vi "InstrumentStudio Screenshot Capture.vi"(8 "error in":errorcluster, 10 "Base File Name (*.bmp)":string="InstrStudio_Screenshot.bmp", 11 "Output Folder to Save Screenshot":path=path "C:/Temp") -> (0 "error out":errorcluster, 3 "Save Image Successful?":bool)   [LabVIEW 2025, in "Screenshot Utility.lvlib"]
doc: "This VI captures a screenshot of the InstrumentStudio window using Windows GDI APIs (works even if hidden).\n\nFor saving the screenshot of InstrumentStudio:\n • Provide a valid output folder and base file name.\n • Ensure InstrumentStudio is running with required SFPs loaded (window must exist).\n • Automatically appends a timestamp to the file name before saving.\n • Works only on Windows; capture fails if the window is not found or title is incorrect."
uses:
  Screenshot Utility.lvlib
  User32.dll
  GDI32.DLL
panel:
  # "This VI captures a screenshot of the InstrumentStudio window using Windows GDI APIs (works even if hidden).\n\nFor saving the screenshot of InstrumentStudio:\n • Provide a valid output folder and base file name.\n • Ensure InstrumentStudio is running with required SFPs loaded (window must exist).\n • Automatically appends a timestamp to the file name before saving.\n • Works only on Windows; capture fails if the window is not found or title is incorrect."
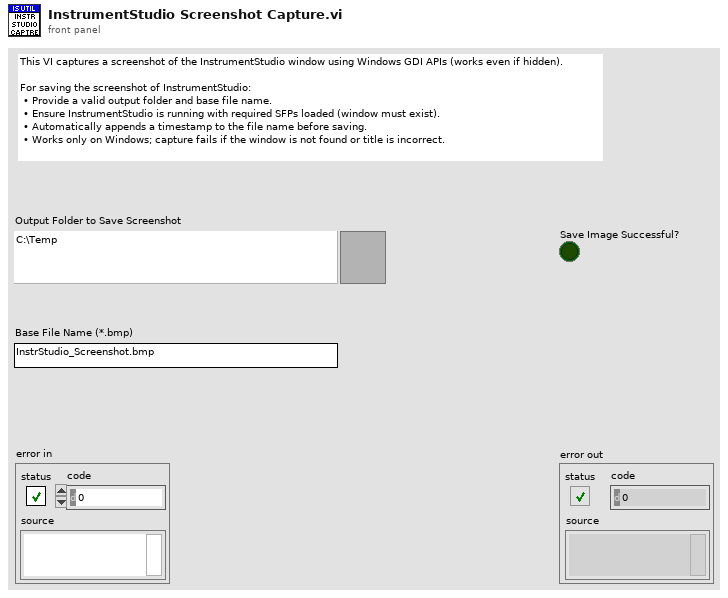
[diagram p1: front panel]
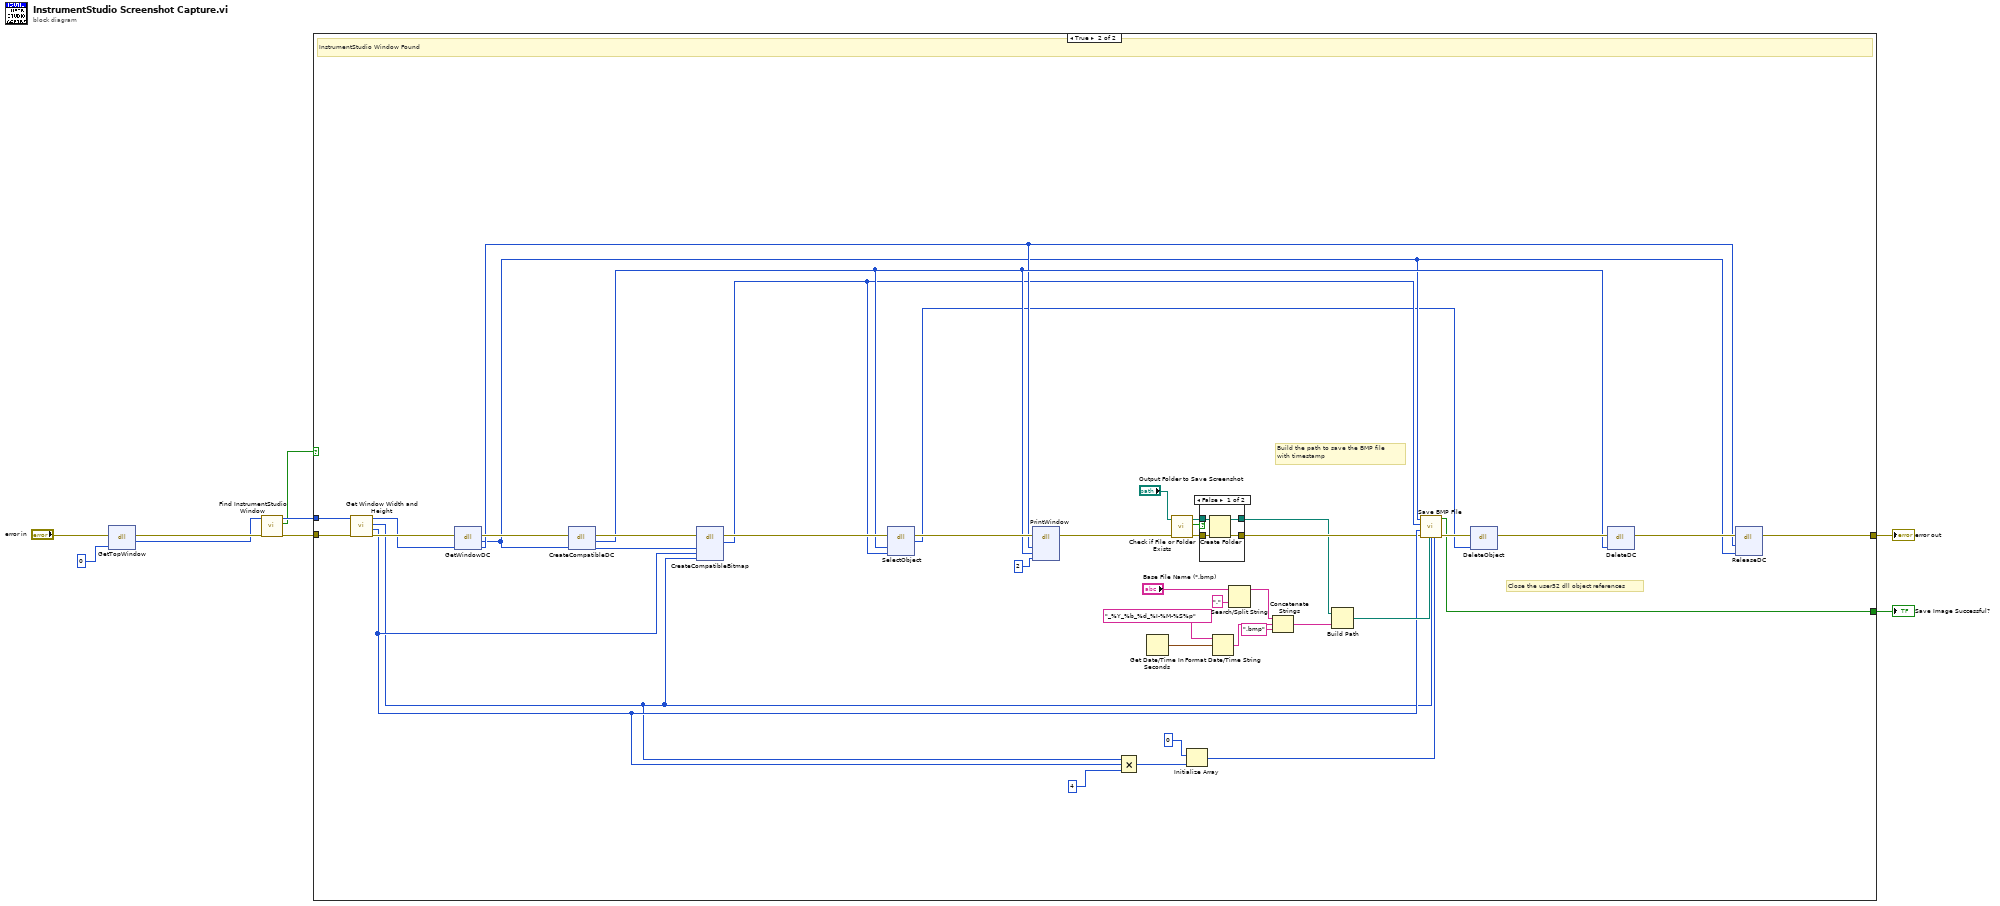
[diagram p0: block diagram]
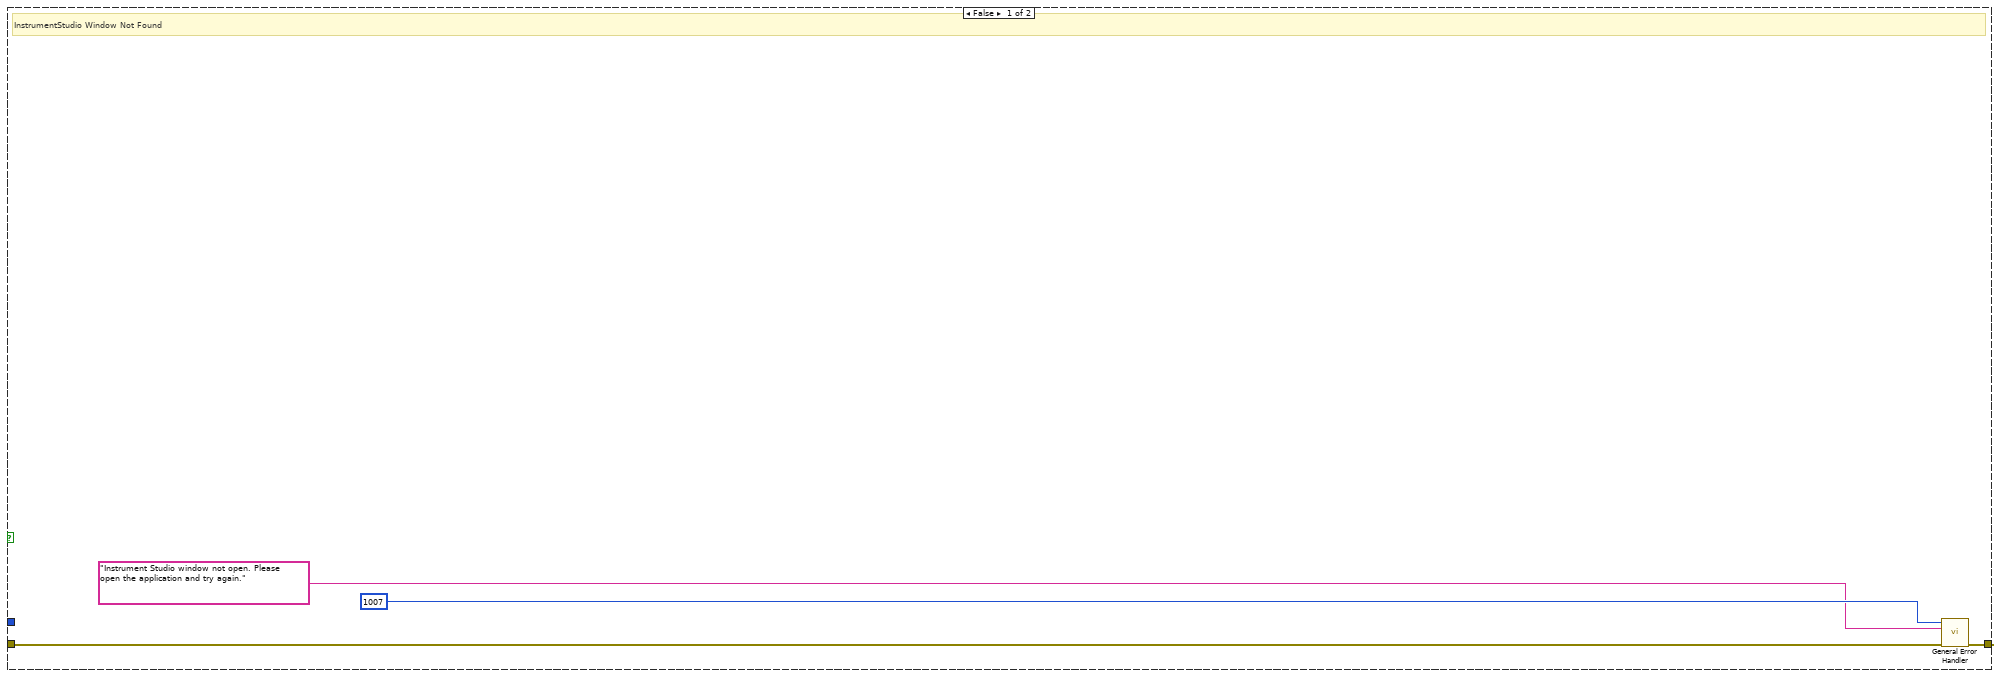
[diagram p2: hidden frame]
diagram:
  n1 = dll-call lib="USER32.DLL" fn="GetTopWindow"(error in="error in", "hWnd"=u32 0) -> (error out=w8:errorcluster, "return"=w6:u32)  [unwired: 2 in, 2 out]
  n2 = call "Find InstrumentStudio Window.vi"("error in"=w8, "Top Window"=w6) -> ("error out"=w3:errorcluster, "IS Window Found?"=w2:bool, "hWnd"=w4:u32)  [unwired: 7 in]
  n3 = case shown="True" w2 {
    tunnel: [w12 w45] -> w5
    tunnel: w4 -> [_ w21]
    tunnel: w3 -> [w13 w22]
    tunnel: [_ w23] -> w1
    frame False {
      # "InstrumentStudio Window Not Found"
      n4 = call <vilib>:"General Error Handler.vi"("[error code] (0)"=1007, "[error source] (\" \")"="Instrument Studio window not open. Please open the application and try again." ("[error source] (\" \")"), "error in (no error)"=w13) -> ("error out"=w12:errorcluster)  [unwired: 8 in, 4 out]
    }
    frame True {
      # "Close the user32 dll object references"
      # "Build the path to save the BMP file \nwith timestamp"
      # "InstrumentStudio Window Found"
      n5 = call "Get Window Width and Height.vi"("error in"=w22, "hWnd in"=w21) -> ("error out"=w41:errorcluster, "Width"=w25:i32, "Height"=w24:i32, "hWnd out"=w39:u32)  [unwired: 6 in]
      n6 = dll-call lib="USER32.DLL" fn="GetWindowDC"(error in=w41, "hWnd"=w39) -> (error out=w55:errorcluster, "return"=w43:u32, "hWnd"=w44:u32)  [unwired: 2 in, 1 out]
      n7 = dll-call lib="GDI32.DLL" fn="CreateCompatibleDC"(error in=w55, "hdc"=w43) -> (error out=w47:errorcluster, "return"=w46:u32, "hdc"=w54:u32)  [unwired: 2 in, 1 out]
      n8 = dll-call lib="GDI32.DLL" fn="CreateCompatibleBitmap"(error in=w47, "hdc"=w54, "cx"=w25, "cy"=w24) -> (error out=w53:errorcluster, "return"=w37:u32)  [unwired: 2 in, 4 out]
      n9 = dll-call lib="GDI32.DLL" fn="SelectObject"(error in=w53, "hdc"=w46, "h"=w37) -> (error out=w52:errorcluster, "return"=w35:u32)  [unwired: 2 in, 3 out]
      n10 = dll-call lib="USER32.DLL" fn="PrintWindow"(error in=w52, "hWnd"=w44, "hdcBlt"=w46, "nFlags"=u32 2) -> (error out=w17:errorcluster)  [unwired: 2 in, 5 out]
      n11 = Compound Arithmetic op=MULTIPLY(w24, w25, 4 ("value")) -> (w42:i32)
      n12 = Get Date/Time In Seconds() -> (seconds since 1Jan1904=w34:timestamp)
      n13 = call <vilib>:"Check if File or Folder Exists.vi"("error in (no error)"=w17, "path"="Output Folder to Save Screenshot") -> ("error out"=w20:errorcluster, "file or folder exists?"=w18:bool, "dup path"=w19:path)  [unwired: 7 in]
      n14 = Initialize Array(u8 0 ("element"), w42) -> (w38:u8[])
      n15 = case shown="False" w18 {
        tunnel: [w59 w60] -> w16
        tunnel: [w58 w61] -> w14
        tunnel: w20 -> [w57 w60]
        tunnel: w19 -> [w56 w61]
        frame False {
          n16 = Create Folder(path (use dialog)=w56, error in=w57) -> (created path=w58:path, error out=w59:errorcluster)  [unwired: 1 in, 1 out]
        }
        frame True {
        }
      }
      n17 = Format Date/Time String(time format string (%c)="_%Y_%b_%d_%I-%M-%S%p", seconds (now)=w34) -> (date/time string=w29:string)  [unwired: 1 in]
      n18 = Search/Split String(string="Base File Name (*.bmp)", search string/char (-)=".") -> (substring before match=w30:string)  [unwired: 1 in, 2 out]
      n19 = Concatenate Strings(w30, w29, ".bmp" ("string")) -> (w27:string)
      n20 = Build Path(base path=w14, name or relative path=w27) -> (appended path=w26:path)
      n21 = call "Save BMP File.vi"("lpvBits Array"=w38, "Height"=w24, "Path to BMP file"=w26, "error in"=w16, "Width"=w25, "hbm"=w37, "hdc"=w43) -> ("error out"=w36:errorcluster, "Save Image Successful?"=w23:bool)  [unwired: 3 in]
      n22 = dll-call lib="GDI32.DLL" fn="DeleteObject"(error in=w36, "hObject"=w35) -> (error out=w49:errorcluster)  [unwired: 2 in, 3 out]
      n23 = dll-call lib="GDI32.DLL" fn="DeleteDC"(error in=w49, "hObject"=w46) -> (error out=w48:errorcluster)  [unwired: 2 in, 3 out]
      n24 = dll-call lib="USER32.DLL" fn="ReleaseDC"(error in=w48, "hWnd"=w44, "hDC"=w43) -> (error out=w45:errorcluster)  [unwired: 2 in, 4 out]
    }
  }
  "error out" <- w5
  "Save Image Successful?" <- w1
